vi "ReadChannelsFile.vi"(8 "error in (no error)":errorcluster, 11 "object in":refnum<class "ChannelsManager.lvclass">) -> (0 "error out":errorcluster, 2 "Channels File":path, 3 "object out":refnum<class "ChannelsManager.lvclass">)   [LabVIEW 2021, in "Channel.lvlib" / "ChannelsManager.lvlib" / "ChannelsManager.lvclass"]
uses:
  ChannelsManager.lvclass
  ChannelsManager.lvclass/ChannelsManager.ctl
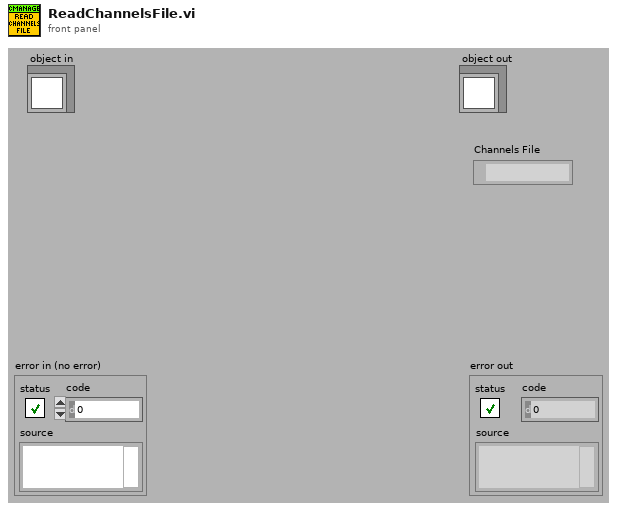
[diagram p1: front panel]
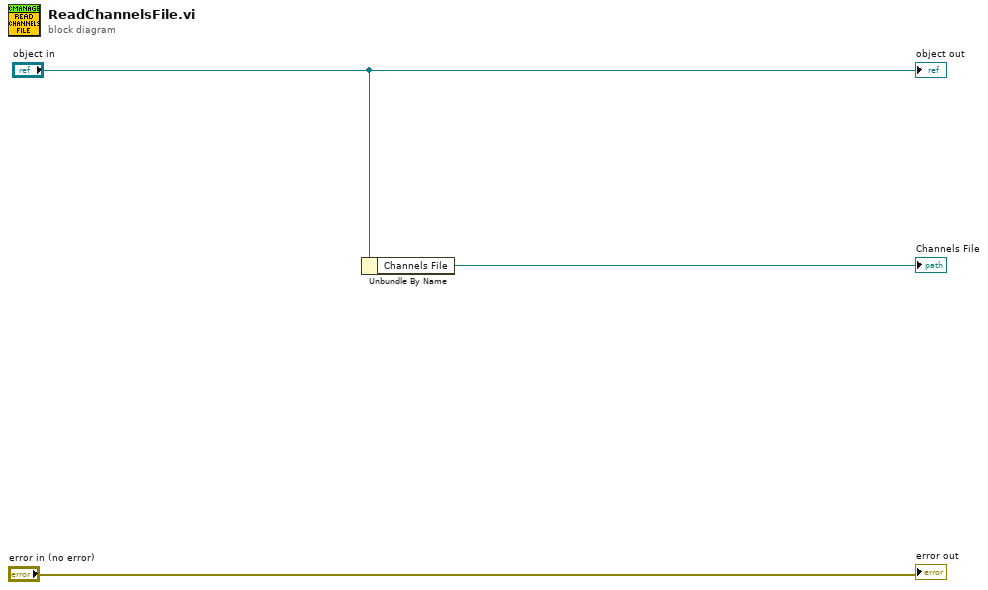
[diagram p0: block diagram]
diagram:
  n1 = Unbundle By Name("object in") -> ("Channels File"=→"Channels File":path)
  "error out" <- "error in (no error)"
  "object out" <- "object in"
